vi "Test selection.vi"(11 "Cluster 2":T1={"Unit Model "="", "Reported by"="", "Test Standard"="", "Tested by"="", "Job Number"="NA", "Test Facility"="40TR-Lab", "Power Supply"="", "Other:    PS"="", "Unit Family"="Package", "Requester"="ENG", "Client "="", "Project"="", "Serial Number"="", "Brand"="", "Manufacturer"="", "Test Type"="Package"}) -> (2 "Selected Tests":string[](array[string]), 3 "subarray":string[](array[string]))   [LabVIEW 2025]
panel:
  out "array w/ subset deleted":string[](array[string])
  out "subarray 3":string[](array[string])
  out "subarray 2":string[](array[string])
  out "x = y?":bool
  in  "String 2":string
  in  "String":string
  out "Unit Family":string
  out "Array":string[](array[string])
  out "Tested by":string
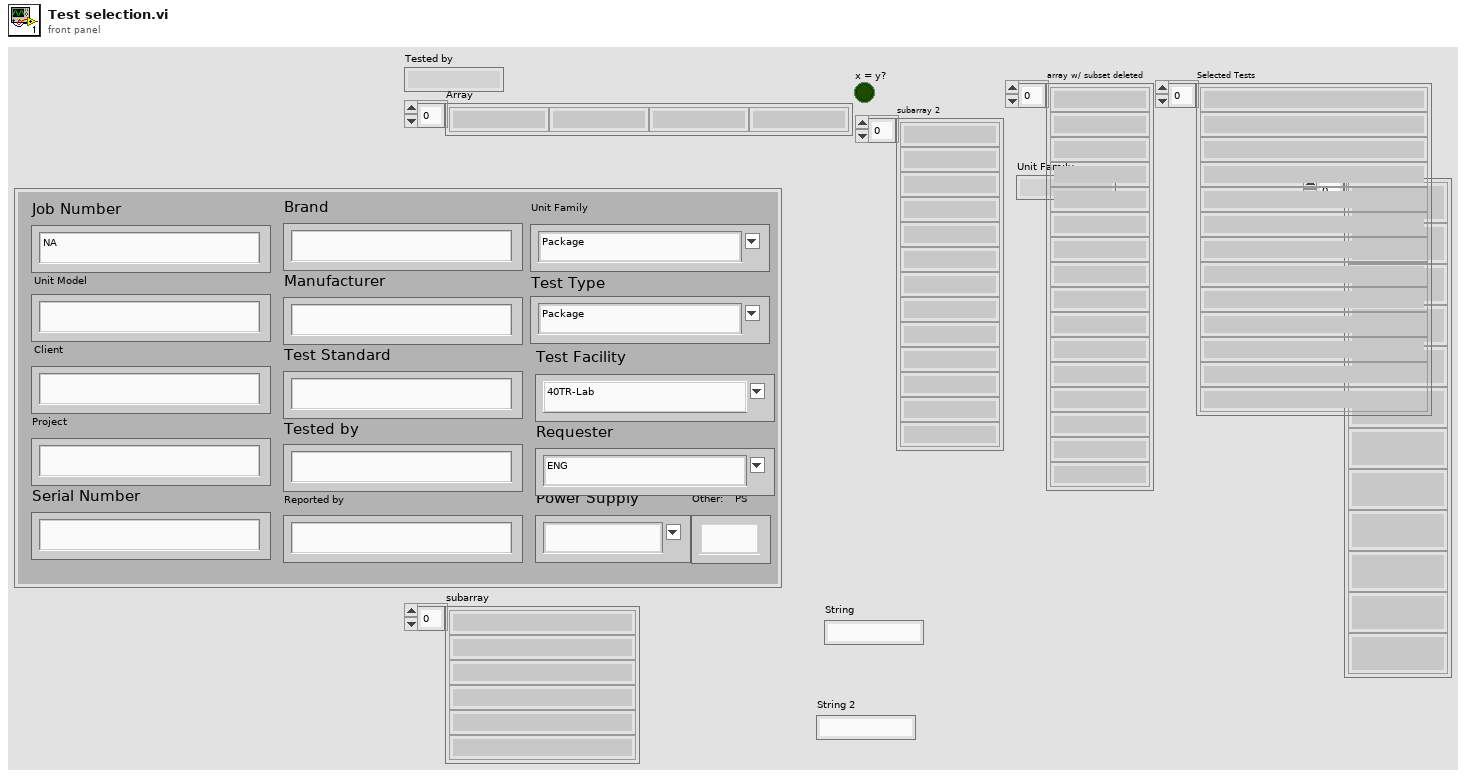
[diagram p1: front panel]
types:
  T1 = cluster{"Unit Model ":string, "Reported by":string, "Test Standard":string, "Tested by":string, "Job Number":string, "Test Facility":string, "Power Supply":string, "Other:    PS":string, "Unit Family":string, "Requester":string, "Client ":string, "Project":string, "Serial Number":string, "Brand":string, "Manufacturer":string, "Test Type":string}
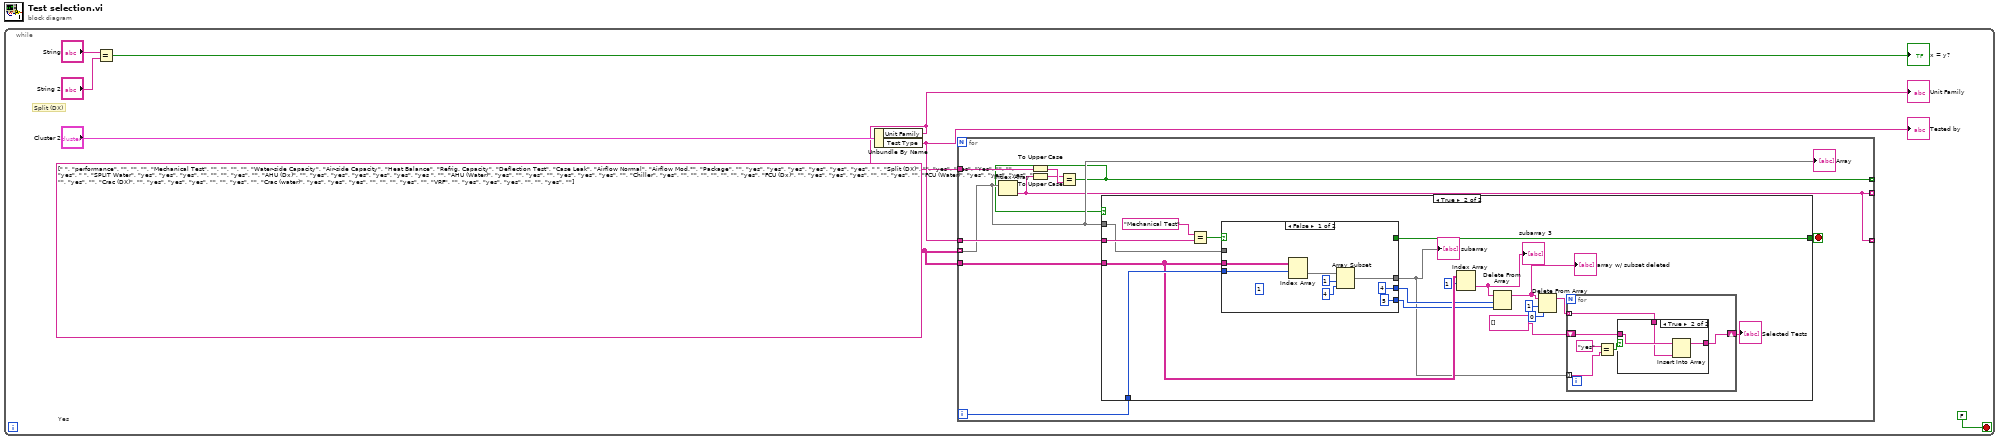
[diagram p0: block diagram]
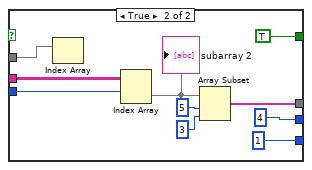
[diagram p4: hidden frame]
diagram:
  n1 = while {
    stop <- FALSE stop-if-true
    w5 = string[][] [[" ", "performance", "", "", "", "Mechanical Test", "", "", ""], ["", "Water-side Capacity", "Air-side Capacity", "Heat Balance", "Refrig. Capacity", "Deflection Test", "Case Leak", "Airflow Normal", "Airflow Mod.*"], ["Package", "", "yes", "yes", "yes", "yes", "yes", "yes", " "], ["Split (DX)", "", "yes", "yes", "Yes", "", "", "yes", " "], ["SPLIT Water", "yes", "yes", "yes", "", "", "", "yes", ""], ["AHU (Dx)", "", "yes", "yes", "yes", "yes", "yes", "yes ", ""], ["AHU (Water)", "yes", "", "yes", "", "yes", "yes", "yes", ""], ["Chiller", "yes", "", "", "", "", "", "", "yes"], ["FCU (Dx)", "", "yes", "yes", "yes", "", "", "yes", ""], ["FCU (Water)", "yes", "yes", "yes", "", "", "", "yes", ""], ["Crac (DX)", "", "yes", "yes", "yes", "", "", "yes", ""], ["Crac (water)", "yes", "yes", "yes", "", "", "", "yes", ""], ["VRF", "", "yes", "yes", "yes", "", "", "yes", ""]]
    # "Split (DX)"
    # "Yes"
    n2 = Equal?(x="String", y="String 2") -> (x = y?=→"x = y?":bool)
    n3 = Unbundle By Name("Cluster 2") -> ("Unit Family"=w4:string, "Test Type"=w6:string)
    "Tested by" <- w6
    "Unit Family" <- w4
    n4 = for {
      tunnel: w5 -> [w17] mode=indexing
      tunnel: w4 -> [w14]
      tunnel: [w10] -> _ mode=indexing
      tunnel: w6 -> [w18]
      tunnel: w5 -> [w16]
      tunnel: [w11] -> _ mode=indexing
      tunnel: [w10] -> _ mode=indexing
      i -> [w9]
      stop <- w15 stop-if-true
      n5 = Index Array(array=w17) -> (element=w10:string)  [unwired: 1 in]
      n6 = To Upper Case(1:w14) -> (0:w13:string)
      n7 = To Upper Case(1:w10) -> (0:w12:string)
      n8 = Equal?(x=w12, y=w13) -> (x = y?=w11:bool)
      n9 = case shown="True" w11 {
        tunnel: w18 -> [_ w35]
        tunnel: w17 -> [_ w33]
        tunnel: w16 -> [_ w30]
        tunnel: [_ w32] -> w15
        tunnel: w9 -> [_ w31]
        frame False {
        }
        frame True {
          n10 = Equal?(x="Mechanical Test", y=w35) -> (x = y?=w34:bool)
          n11 = case shown="False" w34 {
            tunnel: w33 -> [_ w64]
            tunnel: w30 -> [w52 w63]
            tunnel: [_ TRUE] -> w32
            tunnel: [w50 w58] -> w25
            tunnel: w31 -> [w49 w57]
            tunnel: [5 ("index") 1 ("index")] -> w27
            tunnel: [4 ("length") 4 ("length")] -> w26
            frame False {
              (unwired) 1 ("index (row)")
              n12 = Index Array(array=w52, index (row)=w49) -> (element=w54:string[])  [unwired: 1 in]
              n13 = Array Subset(array=w54, index=1, length=4) -> (w50:string[])
            }
            frame True {
              n14 = Index Array(array=w64) -> ()  [unwired: 1 in, 1 out]
              n15 = Index Array(array=w63, index (row)=w57) -> (element=w62:string[])  [unwired: 1 in]
              "subarray 2" <- w62
              n16 = Array Subset(array=w62, index=5, length=3) -> (w58:string[])
            }
          }
          "subarray" <- w25
          n17 = Index Array(array=w30, index (row)=1) -> (element=w28:string[])  [unwired: 1 in]
          "subarray 3" <- w28
          n18 = Delete From Array(array=w28, length=w26, index=w27) -> (array with subset deleted=w22:string[])  [unwired: 1 out]
          "array w/ subset deleted" <- w22
          n19 = Delete From Array(array=w22, length=1, index=0) -> (array with subset deleted=w20:string[])  [unwired: 1 out]
          n20 = for {
            tunnel: w25 -> [w42] mode=indexing
            shift-right: [w39] -> w23
            shift-left: string[] [] -> [w40]
            tunnel: w20 -> [w38] mode=indexing
            n21 = Equal?(x="yes", y=w42) -> (x = y?=w37:bool)
            n22 = case shown="True" w37 {
              tunnel: w40 -> [w43 w46]
              tunnel: [w43 w45] -> w39
              tunnel: w38 -> [_ w44]
              frame False {
              }
              frame True {
                n23 = Insert Into Array(array=w46, new element=w44) -> (w45:string[])  [unwired: 1 in]
              }
            }
          }
          "Selected Tests" <- w23
        }
      }
      "Array" <- w17
    }
  }
